vi "DAC Configure.vi"(8 "error in":errorcluster, 11 "DAC HS Vib in":refnum<class "DAC HS Vib.lvclass">) -> (0 "error out":errorcluster, 3 "DAC HS Vib out":refnum<class "DAC HS Vib.lvclass">)   [LabVIEW 2019, in "DAC.lvlib" / "DAC HS Vib.lvclass"]
uses:
  DAC HS Vib.lvclass
  C:/Users/krio/Documents/LV_Projects/test-stand/App/DAC/DAC.lvclass
  DAC.lvclass/DAC.ctl
  DAC HS Vib.lvclass/DAC HS Vib.ctl
  <vilib>/DAQmx/create/scale.llb/DAQmx Create Scale (Map Ranges).vi
  <vilib>/DAQmx/create/channels.llb/DAQmx Create Channel (AI-Current-Basic).vi
  <vilib>/DAQmx/create/channels.llb/DAQmx Create Channel (AI-Voltage-Basic).vi
  <vilib>/DAQmx/configure/timing.llb/DAQmx Timing (Sample Clock).vi
  DAC.lvclass
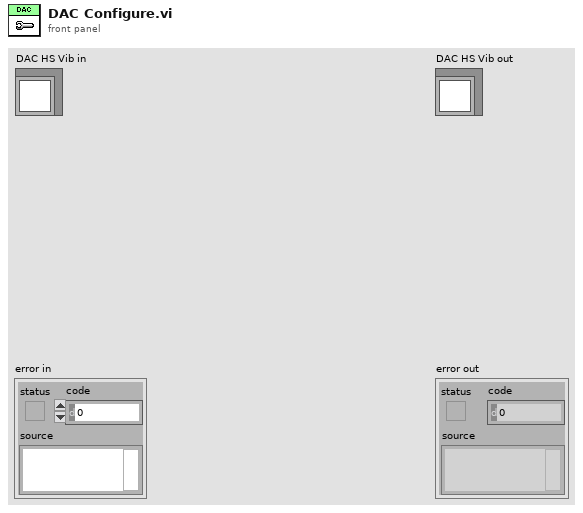
[diagram p1: front panel]
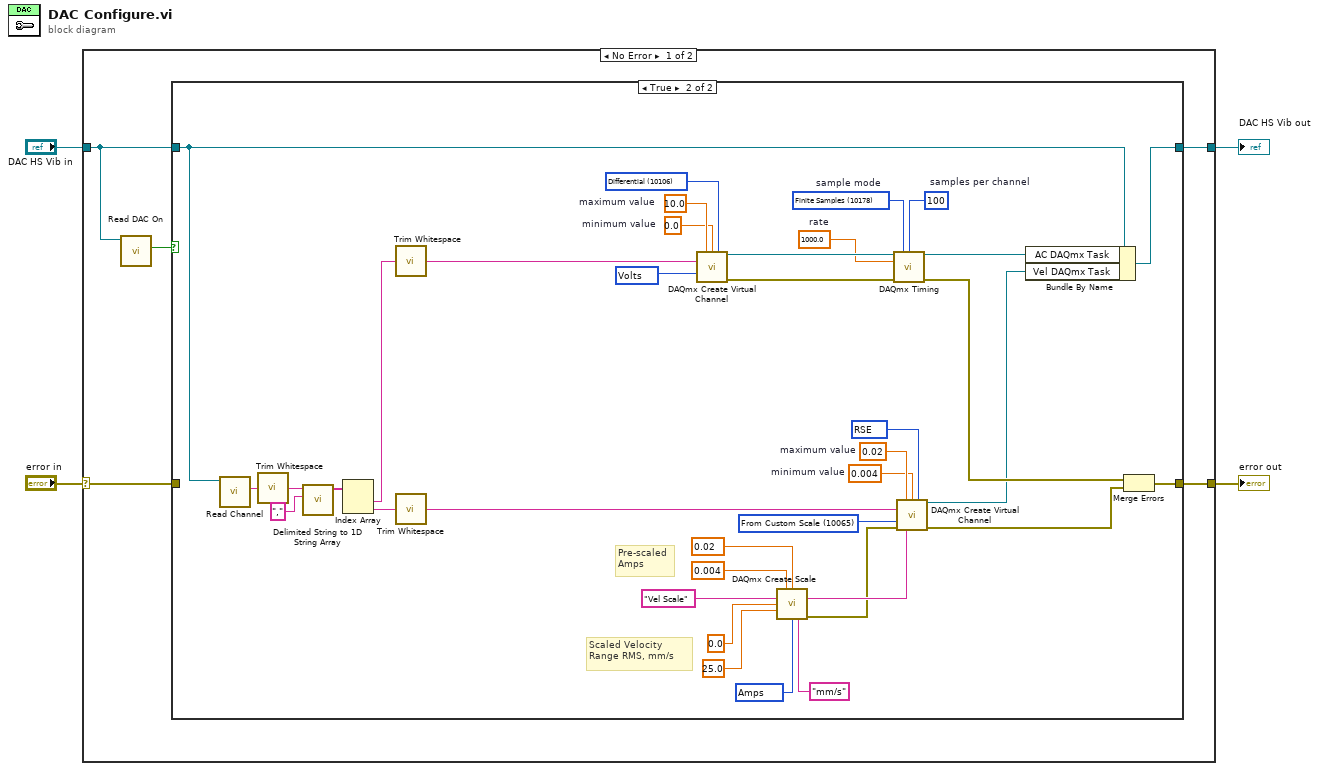
[diagram p0: block diagram]
diagram:
  n1 = case shown="No Error" "error in" {
    selector: "error in" -> [w6 w50]
    tunnel: [w5 w50] -> w4
    tunnel: [w7 w49] -> w3
    tunnel: "DAC HS Vib in" -> [w9 w49]
    frame No Error {
      n2 = call "Read DAC On.vi"("DAC in"=w9) -> ("DAC On"=w8:bool)  [unwired: 8 in, 2 out]
      n3 = case shown="True" w8 {
        tunnel: w9 -> [w11 w14]
        tunnel: [w11 w44] -> w7
        tunnel: w6 -> [w10 _]
        tunnel: [w10 w43] -> w5
        frame False {
        }
        frame True {
          w13 = 10342 items=["Volts"=10348, "Amps"=10342, "Deg F"=10144, "Deg C"=10143, "Deg R"=10145, "Kelvins"=10325, "Strain"=10299, "Ohms"=10384, "Hz"=10373, "Seconds"=10364, "Meters"=10219, "Inches"=10379, "Degrees"=10146, "Radians"=10273, "Ticks"=10304, "g"=10186, "m/s^2"=12470, "m/s"=15959, "in/s"=15960, "Pascals"=10081, "Newtons"=15875, "Pounds"=15876, "kgf"=15877, "psi"=15879, "bar"=15880, "Nm"=15881, "oz-in"=15882, "lb-in"=15883, "lb-ft"=15884, "Volts/Volt"=15896, "mVolts/Volt"=15897, "pCoulombs"=16103, "Coulombs"=16102, "From TEDS"=12516] ("pre-scaled units")
          w27 = 10083 items=["Default"=-1, "RSE"=10083, "NRSE"=10078, "Differential"=10106, "Pseudodifferential"=12529] ("input terminal configuration")
          w28 = 0.004  # minimum value
          w29 = 0.02  # maximum value
          w31 = 10065 items=["Volts"=10348, "From Custom Scale"=10065] ("units")
          w32 = 10106 items=["Default"=-1, "RSE"=10083, "NRSE"=10078, "Differential"=10106, "Pseudodifferential"=12529] ("input terminal configuration")
          w33 = 0.0  # minimum value
          w34 = 10.0  # maximum value
          w35 = 100  # samples per channel
          w36 = 1000.0  # rate
          w37 = 10178 items=["Finite Samples"=10178, "Continuous Samples"=10123, "Hardware Timed Single Point"=12522]  # sample mode
          w40 = 10348 items=["Volts"=10348, "From Custom Scale"=10065] ("units")
          # "Scaled Velocity Range RMS, mm/s"
          # "Pre-scaled\nAmps"
          n4 = call "Read Channel.vi"("DAC in"=w14) -> ("Channel"=w48:string)  [unwired: 8 in, 2 out]
          n5 = call <vilib>:"Trim Whitespace.vi"("string"=w48) -> ("trimmed string"=w46:string)  [unwired: 1 in]
          n6 = call <vilib>:"Delimited String to 1D String Array.vi"("delimiter"=",", "delimited string"=w46) -> ("string array"=w45:string[])  [unwired: 9 in]
          n7 = Index Array(array=w45) -> (element #1=w19:string, element #2=w16:string)  [unwired: 2 in]
          n8 = call <vilib>:"Trim Whitespace.vi"("string"=w19) -> ("trimmed string"=w18:string)  [unwired: 1 in]
          n9 = call <vilib>:"Trim Whitespace.vi"("string"=w16) -> ("trimmed string"=w17:string)  [unwired: 1 in]
          n10 = call-poly <vilib>:"DAQmx Create Virtual Channel.vi"("maximum value"=w34, "minimum value"=w33, "input terminal configuration"=w32, "physical channels"=w18, "units"=w40) -> ("task out"=w39:refnum<k21>, "error out"=w38:errorcluster)  [unwired: 9 in]
          n11 = call-poly <vilib>:"DAQmx Create Scale.vi"("pre-scaled minimum"=0.004, "pre-scaled maximum"=0.02, "name"="Vel Scale", "scaled minimum"=0.0, "scaled maximum"=25.0, "pre-scaled units"=w13, "scaled units"="mm/s") -> ("scale out"=w21:tag, "error out"=w20:errorcluster)  [unwired: 7 in]
          n12 = call-poly <vilib>:"DAQmx Timing.vi"("task/channels in"=w39, "sample mode"=w37, "samples per channel"=w35, "rate"=w36, "error in"=w38) -> ("task out"=w15:refnum<k21>, "error out"=w42:errorcluster)  [unwired: 9 in]
          n13 = call-poly <vilib>:"DAQmx Create Virtual Channel.vi"("maximum value"=w29, "minimum value"=w28, "input terminal configuration"=w27, "physical channels"=w17, "units"=w31, "error in"=w20, "custom scale name"=w21) -> ("task out"=w30:refnum<k21>, "error out"=w41:errorcluster)  [unwired: 7 in]
          n14 = Bundle By Name(cluster=w14, "AC DAQmx Task"=w15, "Vel DAQmx Task"=w30) -> (w44:refnum<class "DAC HS Vib.lvclass">)
          n15 = Merge Errors(w42, w41) -> (w43:errorcluster)
        }
      }
    }
    frame Error {
    }
  }
  "error out" <- w4
  "DAC HS Vib out" <- w3
